vi "FuncVI-SndIn.vi"(5 "InstanceRef":T2, 9 "arg list":T1[](array[typedef]) {"num" format="%.2f"}) -> (0 "error out":bool, 3 "result":T1 {"num" format="%.2f"})   [LabVIEW 2021]
doc: "<B>FuncVI-SndIn</B>\n\nThis VI is example of implementation of CalcExpress function (FuncVI). The function reads sound from a sound input device and returns it as 1D Array of DBL values.\n\n::: CalcExpress Toolkit :::\nCopyright (c) 2000-2026 Konstantin Shifershteyn. All rights reserved."
uses:
  vi.lib/addons/CalcExpress/cetypes.llb/CalcExpress Function Argument Info.ctl
  vi.lib/addons/CalcExpress/cetypes.llb/CalcExpress Instance RefNum.ctl
  <vilib>/sound2/lvsound2.llb/Sampling Mode.ctl
  <vilib>/sound2/lvsound2.llb/Sound Data Format.ctl
  <vilib>/sound2/lvsound2.llb/Sound Input Read (DBL).vi
  <vilib>/Waveform/WDTOps.llb/WDT Index Channel DBL.vi
panel:
  in  "max arg num":i32=3
  in  "min arg num":i32
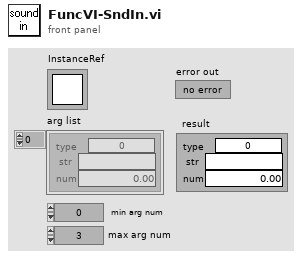
[diagram p1: front panel]
types:
  T1 = typedef "CalcExpress Function Argument Info.ctl" = cluster{"type":u32, "str":string, "num":dbl}
  T2 = typedef "CalcExpress Instance RefNum.ctl" = refnum<k1>
  T3 = enum32{"String", "DBL Number", "identifier", "1D Array of DBL", "2D Array of DBL", "CDB Number", "1D Array of CDB", "2D Array of CDB", "1D Array of String", "2D Array of String", "Unknown data type"}
  T4 = cluster{"index":i32, "data type":enum32{"String", "DBL Number", "identifier", "1D Array of DBL", "2D Array of DBL", "CDB Number", "1D Array of CDB", "2D Array of CDB", "1D Array of String", "2D Array of String", "Unknown data type"}, "default num":dbl, "default str":string}[]
  T5 = typedef "Sound Data Format.ctl" = cluster{"sample rate (S/s)":dbl, "number of channels":i32, "bits per sample":i32}
  T6 = typedef "Sampling Mode.ctl" = i32
  T7 = typedef "Sound Input Task ID.ctl" = u32
  T8 = cluster{"data type":enum32{"String", "DBL Number", "identifier", "1D Array of DBL", "2D Array of DBL", "CDB Number", "1D Array of CDB", "2D Array of CDB", "1D Array of String", "2D Array of String", "Unknown data type"}, "data string":string, dbl}
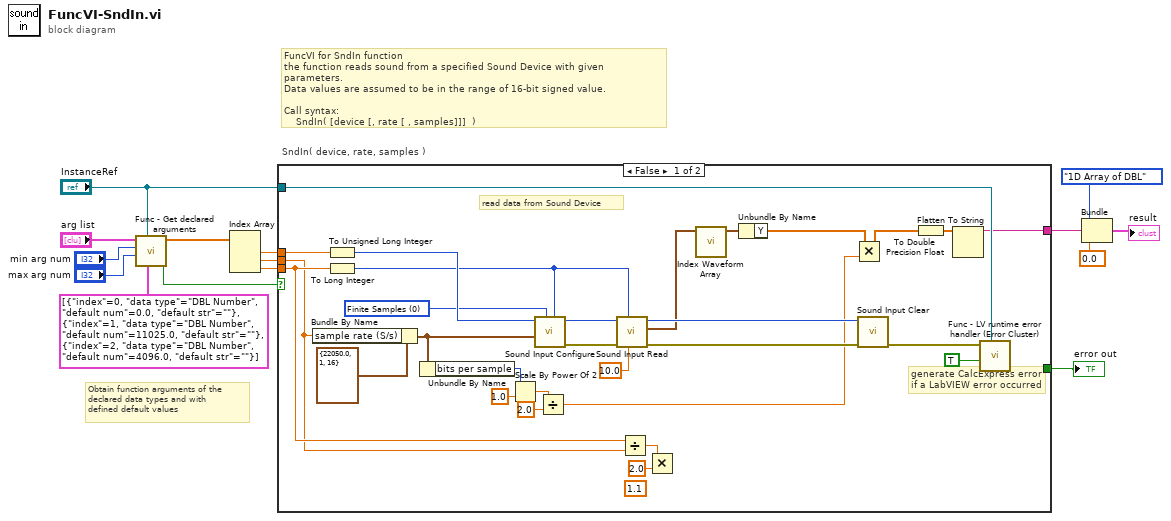
[diagram p0: block diagram]
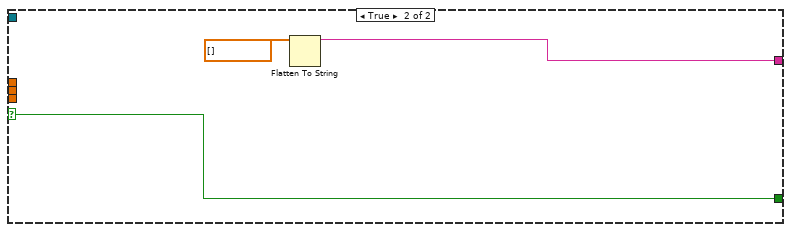
[diagram p2: hidden frame]
diagram:
  # "FuncVI for SndIn function\nthe function reads sound from a specified Sound Device with given parameters.\nData values are assumed to be in the range of 16-bit signed value.\n\nCall syntax:\n    SndIn( [device [, rate [ , samples]]]  )"
  # "Obtain function arguments of the\ndeclared data types and with\ndefined default values"
  # "SndIn( device, rate, samples )"
  n1 = call "Func - Get declared arguments.vi"("arg descriptors"=T4 [{"index"=0, "data type"=enum."DBL Number", "default num"=0.0, "default str"=""}, {"index"=1, "data type"=enum."DBL Number", "default num"=11025.0, "default str"=""}, {"index"=2, "data type"=enum."DBL Number", "default num"=4096.0, "default str"=""}] ("args descriptors"), "InstanceRef"="InstanceRef", "max arg num"="max arg num", "min arg num"="min arg num", "arg list"="arg list") -> ("error out"=w13:bool, "num list"=w1:dbl[])  [unwired: 3 in, 2 out]
  n2 = Index Array(array=w1) -> (element #1=w4:dbl, element #2=w3:dbl, element #3=w2:dbl)  [unwired: 3 in]
  n3 = case shown="False" w13 {
    selector: w13 -> [_ w48]
    tunnel: w3 -> [w25 _]
    tunnel: w2 -> [w26 _]
    tunnel: w4 -> [w45 _]
    tunnel: [w44 w48] -> w12
    tunnel: [w23 w47] -> w11
    tunnel: "InstanceRef" -> [w43 _]
    frame False {
      (unwired) 1.1 ("y")
      w19 = T6 0 items=["Finite Samples", "Continuous Samples"] ("sample mode")
      # "read data from Sound Device"
      # "generate CalcExpress error\nif a LabVIEW error occurred"
      n4 = Bundle By Name(cluster=T5 {"sample rate (S/s)"=22050.0, "number of channels"=1, "bits per sample"=16} ("sound format"), "sample rate (S/s)"=w25) -> (w32:T5)
      n5 = To Unsigned Long Integer(number=w45) -> (unsigned 32bit integer=w33:u32)
      n6 = To Long Integer(number=w26) -> (32bit integer=w17:i32)
      n7 = Unbundle By Name(w32) -> ("bits per sample"=w38:i32)
      n8 = Scale By Power Of 2(n=w38, x=1.0) -> (x*2^n=w37:dbl)
      n9 = call <vilib>:"Sound Input Configure.vi"("number of samples/ch"=w17, "sample mode"=w19, "sound format"=w32, "device ID"=w33) -> ("error out"=w20:errorcluster, "task ID"=w21:T7)  [unwired: 6 in]
      n10 = Divide(x=w37, y=2.0) -> (x/y=w29:dbl)
      n11 = call-poly <vilib>:"Sound Input Read.vi"("timeout (sec)"=10.0, "number of samples/ch"=w17, "error in (no error)"=w20, "task ID"=w21) -> ("error out"=w40:errorcluster, "data"=w31:waveform(dbl)[], "task ID out"=w39:T7)  [unwired: 5 in]
      n12 = Divide(x=w26, y=w25) -> (x/y=w27:dbl)
      n13 = Multiply(x=w27, y=2.0) -> ()  [unwired: 1 out]
      n14 = call-poly <vilib>:"Index Waveform Array.vi"("waveform array"=w31) -> ("waveform"=w30:waveform(dbl))  [unwired: 9 in, 1 out]
      n15 = Unbundle By Name(w30) -> ("Y"=w16:dbl[])
      n16 = Multiply(x=w16, y=w29) -> (x*y=w24:dbl[])
      n17 = call <vilib>:"Sound Input Clear.vi"("error in (no error)"=w40, "task ID"=w39) -> ("error out"=w41:errorcluster)  [unwired: 9 in]
      n18 = To Double Precision Float(number=w24) -> (double precision float=w22:dbl[])
      n19 = Flatten To String(anything=w22) -> (data string=w23:string)  [unwired: 3 in, 2 out]
      n20 = call "Func - LV runtime error handler (Error Cluster).vi"("InstanceRef"=w43, "Gen CE error?"=TRUE, "LabVIEW error"=w41) -> ("error out"=w44:bool)  [unwired: 3 in, 3 out]
    }
    frame True {
      n21 = Flatten To String(anything=dbl[] [] ("double precision float")) -> (data string=w47:string)  [unwired: 3 in, 2 out]
    }
  }
  "error out" <- w12
  n22 = Bundle("data type"=T3."1D Array of DBL", "data string"=w11, 0.0) -> (→"result":T8)  [unwired: 1 in]
